vi "Load UserEvents.vi"(6 "wait for reply (T)":bool=TRUE, 8 "error in":errorcluster, 10 "Run ID":string, 11 "Load From Program Data":bool) -> (0 "error out":errorcluster, 1 "timed out?":bool)   [LabVIEW 2026, in "Replay.lvlib"]
doc: "Loads UserEvents.txt deployed by the extension based on the name of the folder (Run ID).\n\n_____\nCreated using DQMH Framework: Event Scripter 7.1.2.1547."
uses:
  Replay.lvlib
  Load UserEvents Argument--cluster.ctl
  Load UserEvents (Reply Payload)--cluster.ctl
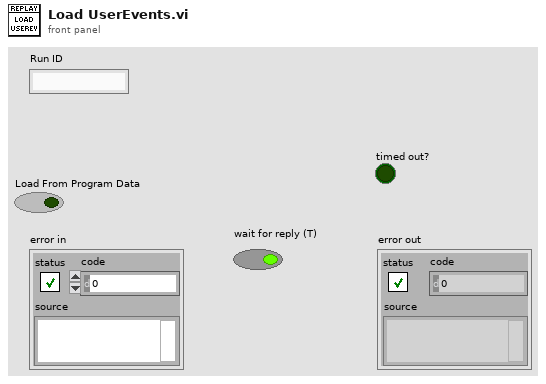
[diagram p1: front panel]
types:
  T1 = typedef "Replay.lvlib/Load UserEvents Argument--cluster.ctl" = cluster{"Run ID":string, "Wait Notifier":refnum<notifier>, "wait for reply":bool, "Load From Program Data":bool}
  T2 = typedef "Replay.lvlib/Request Events--cluster.ctl" = cluster{"Stop Module":refnum<user-event>, "Show Panel":refnum<user-event>, "Hide Panel":refnum<user-event>, "Get Module Execution Status":refnum<user-event>, "Show Diagram":refnum<user-event>, "Set Run ID to Replay":refnum<user-event>, "Load UserEvents":refnum<user-event>, "Private.Trigger Replay Metadata":refnum<user-event>}
  T3 = typedef "Replay.lvlib/Load UserEvents (Reply Payload)--cluster.ctl" = cluster{"error":errorcluster, "Run ID":string, "Load From Program Data":bool}
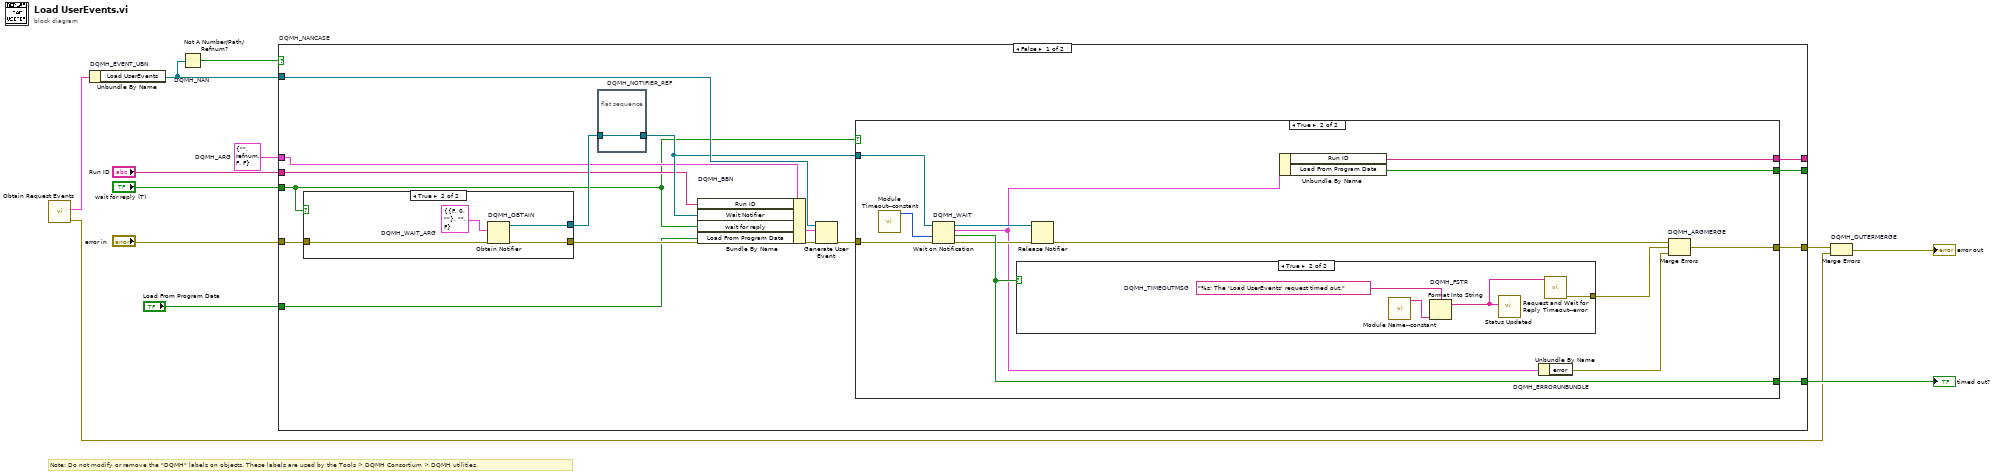
[diagram p0: block diagram]
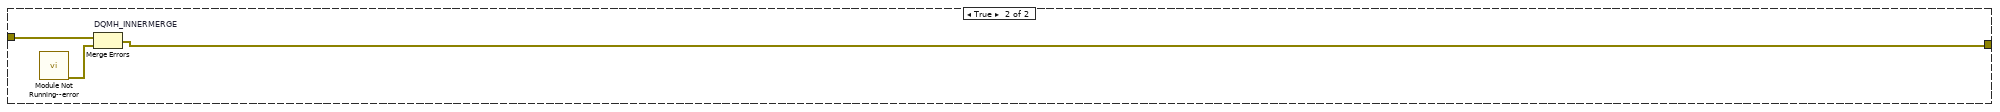
[diagram p5: hidden frame]
diagram:
  w6 = T1 {"Run ID"="", "Wait Notifier"=refnum, "wait for reply"=FALSE, "Load From Program Data"=FALSE}  # DQMH_ARG
  # "Note: Do not modify or remove the \"DQMH\" labels on objects. These labels are used by the Tools > DQMH Consortium > DQMH utilities."
  n1 = call "Obtain Request Events.vi"() -> ("error out"=w3:errorcluster, "Replay Request Events"=w2:T2)  [unwired: 10 in]
  n2 = Unbundle By Name "DQMH_EVENT_UBN"(w2) -> ("Load UserEvents"=w10:refnum<user-event>)
  n3 = Not A Number/Path/Refnum? "DQMH_NAN"(number/path/refnum=w10) -> (NaN/Path/Refnum?=w9:bool)
  n4 = case "DQMH_NANCASE" shown="False" w9 {
    tunnel: "error in" -> [w27 w54]
    tunnel: w10 -> [w25 _]
    tunnel: [w22 w53] -> w7
    tunnel: [w23 _] -> w8
    tunnel: w6 -> [w18 _]
    tunnel: "Run ID" -> [w17 _]
    tunnel: "wait for reply (T)" -> [w16 _]
    tunnel: [w15 _] -> _
    tunnel: [w14 _] -> _
    tunnel: "Load From Program Data" -> [w13 _]
    frame False {
      n5 = case shown="True" w16 {
        tunnel: w27 -> [w47 w51]
        tunnel: [w47 w50] -> w24
        tunnel: [_ w48] -> w20
        frame False {
        }
        frame True {
          w49 = T3 {"error"={"status"=FALSE, "code"=0, "source"=""}, "Run ID"="", "Load From Program Data"=FALSE}  # DQMH_WAIT_ARG
          n6 = Obtain Notifier "DQMH_OBTAIN"(notification data type=w49, error in (no error)=w51) -> (notifier out=w48:refnum<notifier>, error out=w50:errorcluster)  [unwired: 2 in, 1 out]
        }
      }
      n7 = flat-sequence "DQMH_NOTIFIER_REF" {
        tunnel: w20 -> [w28]
        tunnel: [w28] -> w19
        frame #0 {
        }
      }
      n8 = Bundle By Name "DQMH_BBN"(cluster=w18, "Run ID"=w17, "Wait Notifier"=w19, "wait for reply"=w16, "Load From Program Data"=w13) -> (w21:T1)
      n9 = Generate User Event(user event=w25, event data cluster=w21, error in=w24) -> (error out=w26:errorcluster)  [unwired: 1 in, 1 out]
      n10 = case shown="True" w16 {
        tunnel: w26 -> [w29 w42]
        tunnel: w19 -> [_ w41]
        tunnel: [_ w39] -> w23
        tunnel: [w29 w38] -> w22
        tunnel: [_ w31] -> w15
        tunnel: [_ w30] -> w14
        frame False {
        }
        frame True {
          n11 = call "Module Timeout--constant.vi"() -> ("Module Timeout"=w33:i32)  [unwired: 11 in]
          n12 = Wait on Notification "DQMH_WAIT"(notifier=w41, timeout in ms (-1)=w33, error in (no error)=w42) -> (notifier out=w40:refnum<notifier>, notification=w32:T3, timed out?=w39:bool, error out=w37:errorcluster)  [unwired: 1 in]
          n13 = case shown="True" w39 {
            tunnel: [_ w44] -> w34
            frame False {
            }
            frame True {
              w46 = "%s: The 'Load UserEvents' request timed out."  # DQMH_TIMEOUTMSG
              n14 = call "Module Name--constant.vi"() -> ("Module Name"=w43:string)  [unwired: 11 in]
              n15 = Format Into String "DQMH_FSTR"(format string=w46, w43) -> (resulting string=w45:string)  [unwired: 2 in, 1 out]
              n16 = call "Status Updated.vi"("Status"=w45) -> ()  [unwired: 10 in, 1 out]
              n17 = call "Request and Wait for Reply Timeout--error.vi"("Error Message"=w45) -> ("error out"=w44:errorcluster)  [unwired: 10 in]
            }
          }
          n18 = Release Notifier(notifier=w40, error in (no error)=w37) -> (error out=w36:errorcluster)  [unwired: 1 in, 2 out]
          n19 = Unbundle By Name(w32) -> ("Run ID"=w31:string, "Load From Program Data"=w30:bool)
          n20 = Unbundle By Name "DQMH_ERRORUNBUNDLE"(w32) -> ("error"=w35:errorcluster)
          n21 = Merge Errors "DQMH_ARGMERGE"(w36, w34, w35) -> (w38:errorcluster)
        }
      }
    }
    frame True {
      n22 = call "Module Not Running--error.vi"() -> ("error out"=w52:errorcluster)  [unwired: 11 in]
      n23 = Merge Errors "DQMH_INNERMERGE"(w54, w52) -> (w53:errorcluster)
    }
  }
  "timed out?" <- w8
  n24 = Merge Errors "DQMH_OUTERMERGE"(w7, w3) -> (→"error out":errorcluster)
